vi "VIH ProjFile - Product Info - Read.vi"(8 "error in":errorcluster, 11 "XML Parent Item":refnum<k20>) -> (0 "error out":errorcluster, 1 "Product Info out":T1, 3 "dup XML Parent Item":refnum<k20>)   [LabVIEW 2014]
doc: "::: VI Helpeks :::\nCopyright (c) 2000-2026 Konstantin Shifershteyn. All rights reserved."
uses:
  _VIH HelpGen.llb/VIH HelpGen Typedef - Product Info Cluster.ctl
  <vilib>/xml/Close Reference(Node).vi
  <vilib>/xml/NI_XML.lvlib
panel:
  in  "Product Info (data)":T1
  # "VI Helpeks\nCopyright (c) 2012-2026 Konstantin Shifershteyn"
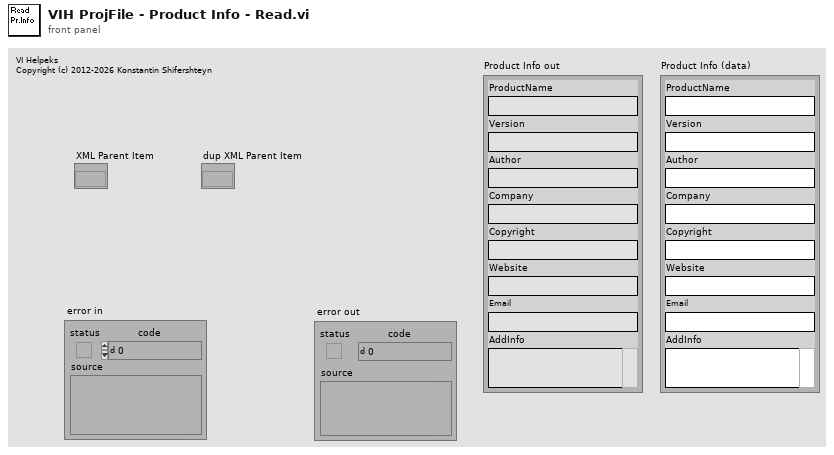
[diagram p1: front panel]
types:
  T1 = typedef "VIH HelpGen Typedef - Product Info Cluster.ctl" = cluster{"ProductName":string, "Version":string, "Author":string, "Company":string, "Copyright":string, "Website":string, "Email":string, "AddInfo":string}
  T2 = typedef "KS HelpGen Typedef - Product Info Cluster.ctl" = cluster{"ProductName":string, "Version":string, "Author":string, "Company":string, "Copyright":string, "Website":string, "Email":string, "AddInfo":string}
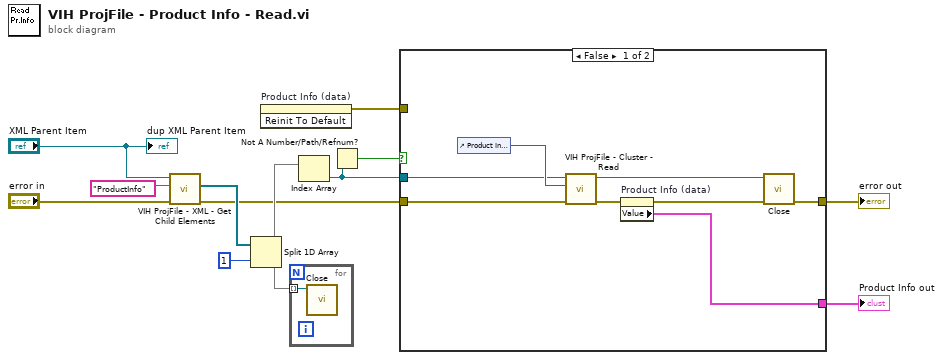
[diagram p0: block diagram]
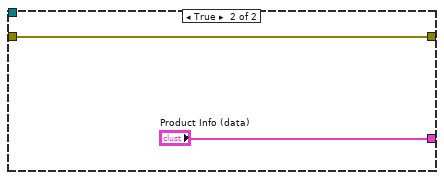
[diagram p2: hidden frame]
diagram:
  n1 = call "VIH ProjFile - XML - Get Child Elements.vi"("error in"="error in", "Tag Name"="ProductInfo", "XML Parent Item"="XML Parent Item") -> ("error out"=w3:errorcluster, "Array of Elements"=w6:refnum<k20>[])  [unwired: 6 in, 1 out]
  n2 = Split 1D Array(array=w6, index=1) -> (first subarray=w9:refnum<k20>[], second subarray=w8:refnum<k20>[])
  n3 = invoke on="Product Info (data)" class="Clust (strict)" method="Reinit To Default"() -> (error out=w2:errorcluster)  [unwired: 3 in, 2 out]
  n4 = for {
    tunnel: w8 -> [w14] mode=indexing
    n5 = call-poly <vilib>:"Close.vi"("node"=w14) -> ()  [unwired: 8 in, 1 out]
  }
  n6 = Index Array(array=w9) -> (element=w12:refnum<k20>)  [unwired: 1 in]
  n7 = Not A Number/Path/Refnum?(number/path/refnum=w12) -> (NaN/Path/Refnum?=w11:bool)
  n8 = case shown="False" w11 {
    tunnel: w3 -> [w15 w24]
    tunnel: [w21 w24] -> w13
    tunnel: [w16 "Product Info (data)"] -> w1
    tunnel: w12 -> [w19 _]
    tunnel: w2 -> [_ _]
    frame False {
      n9 = control-ref of="Product Info (data)"() -> (w22:refnum<vi>)
      n10 = call "VIH ProjFile - Cluster - Read.vi"("error in"=w15, "Ctl Refnum"=w22, "XML Parent Item"=w19) -> ("error out"=w20:errorcluster, "dup XML Parent Item"=w18:refnum<k20>)  [unwired: 7 in]
      n11 = property on="Product Info (data)" class="Clust (strict)"(error in=w20) -> (error out=w17:errorcluster, "Value"=w16:T2)  [unwired: 1 in, 1 out]
      n12 = call-poly <vilib>:"Close.vi"("error in (no error)"=w17, "node"=w18) -> ("error out"=w21:errorcluster)  [unwired: 7 in]
    }
    frame True {
    }
  }
  "error out" <- w13
  "Product Info out" <- w1
  "dup XML Parent Item" <- "XML Parent Item"
